vi "Func - Get DBL argument as 1D Array.vi"(6 "permissions":T1={"scalar enabled"=TRUE, "1d array enabled"=TRUE, "2d array enabled"=TRUE}, 7 "InstanceRef":T3, 8 "error in":bool, 9 "max arg num":i32=1000, 10 "arg idx":i32, 11 "arg list":T4[](array[typedef])) -> (0 "error out":bool, 1 "category":T2(ring), 2 "1D data":dbl[](array[numeric]), 4 "arg type":T5=enum."DBL Number")   [LabVIEW 2021]
doc: "This VI returns the value of a function argument transformed into <b>1D array of DBL</b> values. The requested argument must be a DBL scalar, or a 1D or 2D array thereof. Refer to the VI help for more details.\n\n<b>arg list</b> specifies the list of function arguments passed to a FuncVI. Wire it to the same terminal on the FuncVI block diagram.\n\n<b>arg idx</b> specifies the index of the desired argument.\n\n<b>max arg num</b> specifies the maximum number of arguments.\n\n::: CalcExpress Toolkit :::\nCopyright (c) 2000-2026 Konstantin Shifershteyn. All rights reserved."
uses:
  cetypes.llb/CalcExpress Data Type.ctl
  cetypes.llb/CalcExpress Function Argument Info.ctl
  cetypes.llb/CalcExpress Instance RefNum.ctl
panel:
  out "size(s)":i32[](array[numeric])
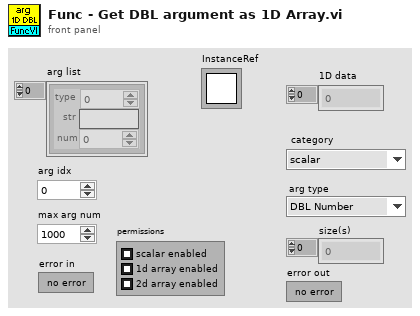
[diagram p1: front panel]
types:
  T1 = cluster{"scalar enabled":bool, "1d array enabled":bool, "2d array enabled":bool}
  T2 = enum16{"scalar", "1D array", "2D array", "ERROR"}
  T3 = typedef "CalcExpress Instance RefNum.ctl" = refnum<k1>
  T4 = typedef "CalcExpress Function Argument Info.ctl" = cluster{"type":u32, "str":string, "num":dbl}
  T5 = typedef "CalcExpress Data Type.ctl" = enum32{"String", "DBL Number", "identifier", "1D Array of DBL", "2D Array of DBL", "CDB Number", "1D Array of CDB", "2D Array of CDB", "1D Array of String", "2D Array of String", "Unknown data type"}
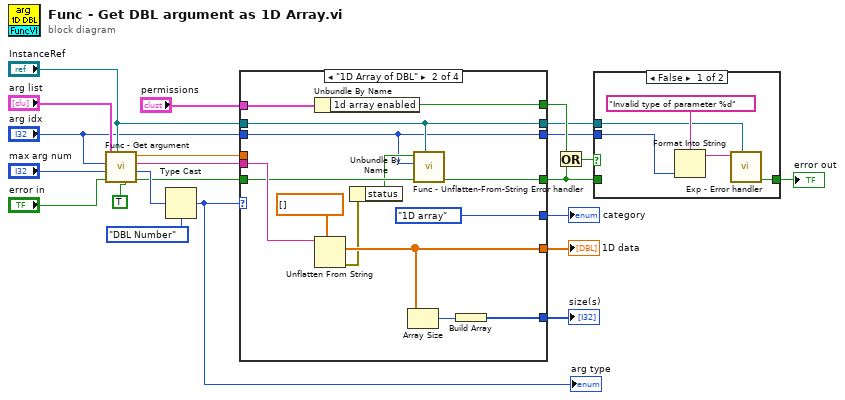
[diagram p0: block diagram]
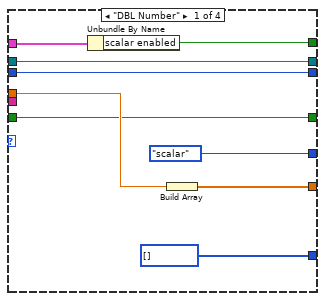
[diagram p3: hidden frame]
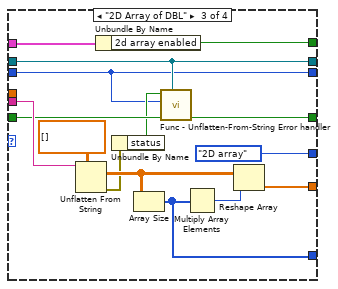
[diagram p4: hidden frame]
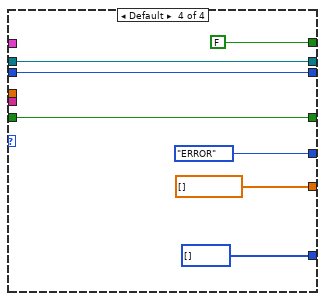
[diagram p5: hidden frame]
diagram:
  n1 = call "Func - Get argument.vi"("ena NonNum? (F)"=TRUE ("ena complex? (F)"), "InstanceRef"="InstanceRef", "error in"="error in", "max arg num"="max arg num", "arg idx"="arg idx", "arg list"="arg list") -> ("error out"=w12:bool, "type"=w16:u32, "str"=w20:string, "num"=w19:dbl)
  n2 = Type Cast(type=CalcExpress_Data_Type."DBL Number" ("data type"), x=w16) -> (*(type *) &x=w14:T5)
  "arg type" <- w14
  n3 = case shown="\"1D Array of DBL\"" w14 {
    tunnel: w20 -> [_ w45 w60 _]
    tunnel: w19 -> [w31 _ _ _]
    tunnel: [w30 w37 w58 dbl[] [] ("2D CDB")] -> w13
    tunnel: w12 -> [w29 w43 w56 w64]
    tunnel: "InstanceRef" -> [w24 w34 w50 w62]
    tunnel: [w29 w42 w54 w64] -> w6
    tunnel: "arg idx" -> [w23 w33 w49 w61]
    tunnel: [T2."scalar" ("category") T2."1D array" ("category") T2."2D array" ("category") T2."ERROR" ("category")] -> w9
    tunnel: [i32[] [] w39 w48 i32[] []] -> w8
    tunnel: "permissions" -> [w26 w36 w52 _]
    tunnel: [w25 w35 w51 FALSE ("2d array enabled")] -> w3
    tunnel: [w24 w34 w50 w62] -> w2
    tunnel: [w23 w33 w49 w61] -> w1
    frame "DBL Number" {
      n4 = Unbundle By Name(w26) -> ("scalar enabled"=w25:bool)
      n5 = Build Array(w31) -> (w30:dbl[])
    }
    frame "1D Array of DBL" {
      n6 = Unbundle By Name(w36) -> ("1d array enabled"=w35:bool)
      n7 = Unflatten From String(type=dbl[] [], binary string=w45) -> (value=w37:dbl[], error out=w32:errorcluster)  [unwired: 3 in, 1 out]
      n8 = Unbundle By Name(w32) -> ("status"=w41:bool)
      n9 = Array Size(array=w37) -> (size(s)=w38:i32)
      n10 = call "Func - Unflatten-From-String Error handler.vi"("InstanceRef"=w34, "error in"=w43, "argument number"=w33, "Unflatten Error status"=w41) -> ("error out"=w42:bool)  [unwired: 5 in]
      n11 = Build Array(w38) -> (w39:i32[])
    }
    frame "2D Array of DBL" {
      n12 = Unflatten From String(type=dbl[][] [], binary string=w60) -> (value=w57:dbl[][], error out=w46:errorcluster)  [unwired: 3 in, 1 out]
      n13 = Unbundle By Name(w52) -> ("2d array enabled"=w51:bool)
      n14 = Unbundle By Name(w46) -> ("status"=w55:bool)
      n15 = Array Size(array=w57) -> (size(s)=w48:i32[])
      n16 = call "Func - Unflatten-From-String Error handler.vi"("InstanceRef"=w50, "error in"=w56, "argument number"=w49, "Unflatten Error status"=w55) -> ("error out"=w54:bool)  [unwired: 5 in]
      n17 = Multiply Array Elements(1:w48) -> (0:w47:i32)
      n18 = Reshape Array(w57, w47) -> (w58:dbl[])
    }
    frame Default {
    }
  }
  "1D data" <- w13
  "category" <- w9
  "size(s)" <- w8
  n19 = Or(x=w3, y=w6) -> (x .or. y?=w7:bool)
  n20 = case shown="False" w7 {
    tunnel: [w70 w73] -> w5
    tunnel: w6 -> [_ w73]
    tunnel: w2 -> [w69 _]
    tunnel: w1 -> [w68 _]
    frame False {
      n21 = Format Into String(format string="Invalid type of parameter %d" ("ErrStr"), w68) -> (resulting string=w71:string)  [unwired: 2 in, 1 out]
      n22 = call "Exp - Error handler.vi"("InstanceRef"=w69, "error message in"=w71) -> ("error out"=w70:bool)  [unwired: 7 in, 2 out]
    }
    frame True {
    }
  }
  "error out" <- w5
